vi "RPC Method ThermalChamberController StopModule.vi"(8 "error in (no error)":errorcluster, 11 "gRPC service in":refnum<class "ThermalChamberController.lvclass">) -> (0 "error out":errorcluster, 3 "gRPC service out":refnum<class "ThermalChamberController.lvclass">)   [LabVIEW 2020, in "thermal-chamber-controller_server.lvlib" / "ThermalChamberController.lvclass"]
uses:
  ThermalChamberController.lvclass
  ThermalChamberController.lvclass/ThermalChamberController.ctl
  Program Files (x86)/National Instruments/LabVIEW 2020/examples/DQMH Consortium/DQMH Fundamentals - Thermal Chamber/Libraries/Thermal Chamber Controller_DQMH/Thermal Chamber Controller_DQMH.lvlib
  RPC Messages/lv_python_grpc_webui_demo_v1_Empty.ctl
  thermal-chamber-controller_server.lvlib
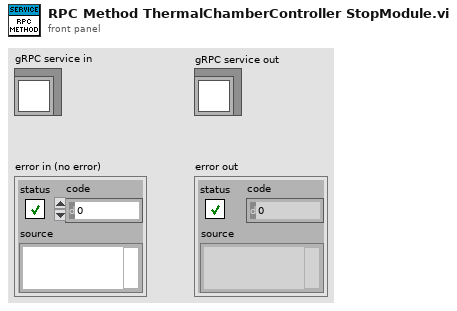
[diagram p1: front panel]
types:
  T1 = typedef "thermal-chamber-controller_server.lvlib/lv_python_grpc_webui_demo_v1_Empty.ctl" = cluster{"void":string}
  T2 = typedef "thermal-chamber-controller_server.lvlib/ThermalChamberController.lvclass/Server Internal UEs.ctl" = cluster{"ThermalChamberController StartModule Internal UE":refnum<user-event>, "ThermalChamberController ShowModulePanel Internal UE":refnum<user-event>, "ThermalChamberController HideModulePanel Internal UE":refnum<user-event>, "ThermalChamberController StopModule Internal UE":refnum<user-event>, "ThermalChamberController UpdateSetPoint Internal UE":refnum<user-event>, "ThermalChamberController UpdateRampRate Internal UE":refnum<user-event>, "ThermalChamberController UpdateHeaterState Internal UE":refnum<user-event>, "ThermalChamberController SubscribeChamberStatusUpdated Internal UE":refnum<user-event>, "ThermalChamberController SubscribeSetPointUpdated Internal UE":refnum<user-event>, "ThermalChamberController SubscribeRampRateUpdated Internal UE":refnum<user-event>, "ThermalChamberController SubscribeHeaterStateUpdated Internal UE":refnum<user-event>}
  T3 = typedef "thermal-chamber-controller_server.lvlib/ThermalChamberController.lvclass/Server gRPC UEs.ctl" = cluster{"ThermalChamberController StartModule gRPC UE":refnum<user-event>, "ThermalChamberController ShowModulePanel gRPC UE":refnum<user-event>, "ThermalChamberController HideModulePanel gRPC UE":refnum<user-event>, "ThermalChamberController StopModule gRPC UE":refnum<user-event>, "ThermalChamberController UpdateSetPoint gRPC UE":refnum<user-event>, "ThermalChamberController UpdateRampRate gRPC UE":refnum<user-event>, "ThermalChamberController UpdateHeaterState gRPC UE":refnum<user-event>, "ThermalChamberController SubscribeChamberStatusUpdated gRPC UE":refnum<user-event>, "ThermalChamberController SubscribeSetPointUpdated gRPC UE":refnum<user-event>, "ThermalChamberController SubscribeRampRateUpdated gRPC UE":refnum<user-event>, "ThermalChamberController SubscribeHeaterStateUpdated gRPC UE":refnum<user-event>}
  T4 = typedef "grpc-lvsupport-release.lvlib/grpcId.ctl" = u64
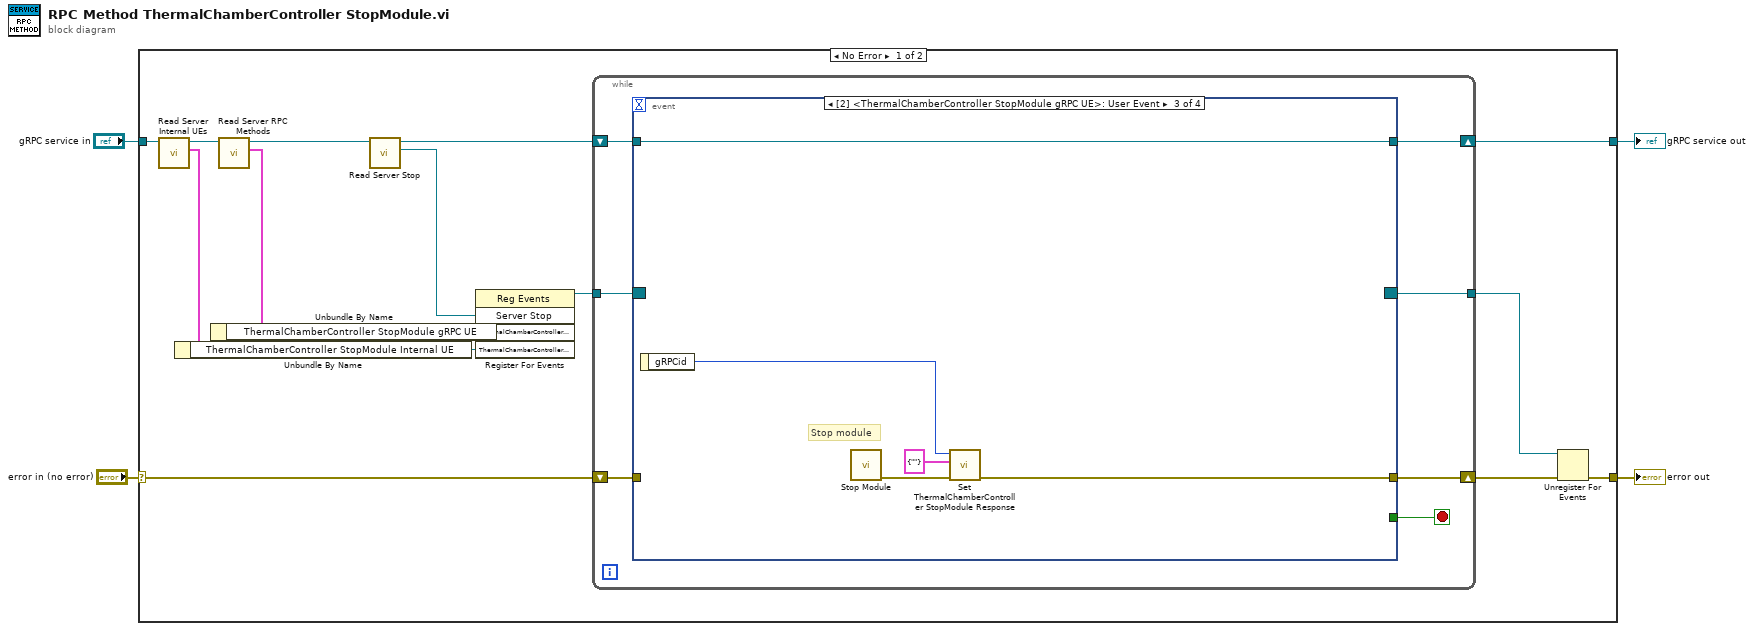
[diagram p0: block diagram]
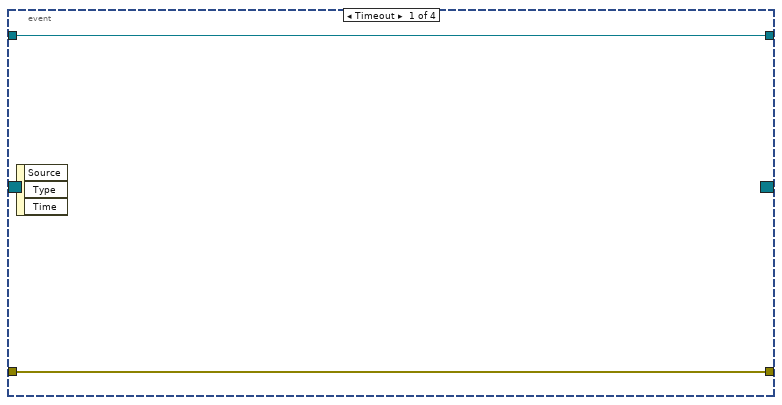
[diagram p2: hidden frame]
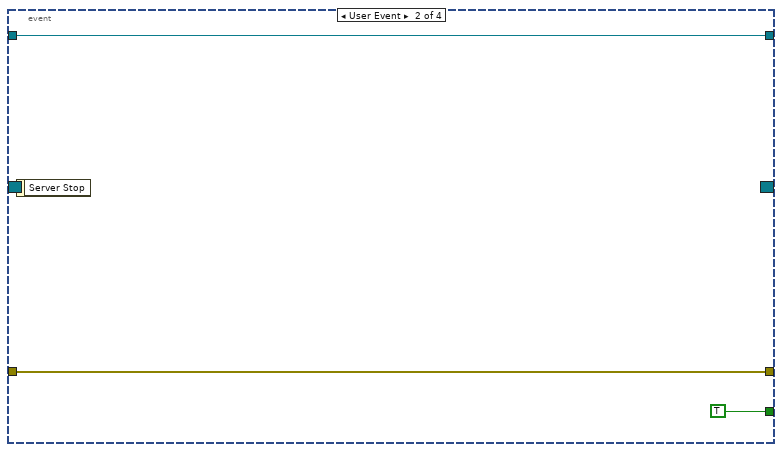
[diagram p3: hidden frame]
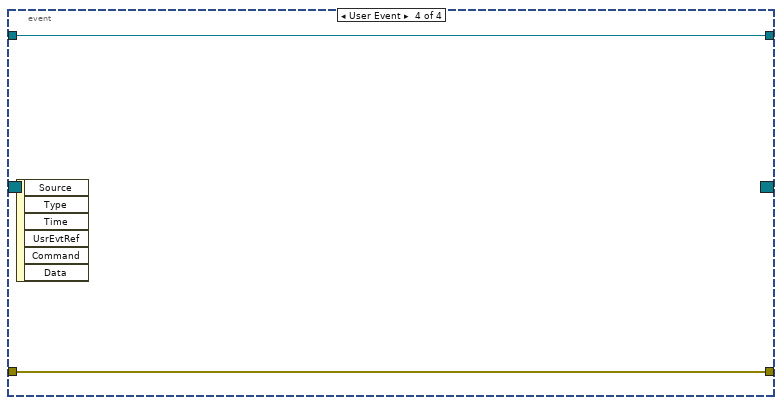
[diagram p4: hidden frame]
diagram:
  n1 = case shown="No Error" "error in (no error)" {
    selector: "error in (no error)" -> [w15 w40]
    tunnel: [w13 w40] -> w3
    tunnel: "gRPC service in" -> [w17 w39]
    tunnel: [w5 w39] -> w1
    frame No Error {
      n2 = call "Read Server Internal UEs.vi"("gRPC service in"=w17) -> ("Server Internal UEs"=w9:T2, "gRPC service out"=w16:refnum<class "ThermalChamberController.lvclass">)  [unwired: 8 in, 1 out]
      n3 = Unbundle By Name ("Unbundle Internal UE")(w9) -> ("ThermalChamberController StopModule Internal UE"=w8:refnum<user-event>)
      n4 = call "Read Server RPC Methods.vi"("gRPC service in"=w16) -> ("Server RPC Methods"=w11:T3, "gRPC service out"=w6:refnum<class "ThermalChamberController.lvclass">)  [unwired: 8 in, 1 out]
      n5 = Unbundle By Name ("Unbundle gRPC UE")(w11) -> ("ThermalChamberController StopModule gRPC UE"=w10:refnum<user-event>)
      n6 = call-dynamic "Read Server Stop.vi"("gRPC service in"=w6) -> ("Server Stop"=w19:refnum<user-event>, "gRPC service out"=w7:refnum<class "ThermalChamberController.lvclass">)  [unwired: 8 in, 1 out]
      n7 = register-events(w19, w10, w8) -> (reference out=w18:refnum<event-registration>)  [unwired: 2 in, 1 out]
      n8 = while {
        tunnel: w18 -> [w26]
        tunnel: [w22] -> w12
        shift-right: [w23] -> w14
        shift-left: w15 -> [w24]
        shift-right: [w20] -> w5
        shift-left: w7 -> [w21]
        stop <- w25 stop-if-true
        n9 = event "RPC Method Event Structure" shown="[2] <ThermalChamberController StopModule gRPC UE>: User Event" {
          selector: w26 -> [_ _ _ _]
          dyn-events: [_ _ _ _] -> w22
          timeout: _ -> [_ _ _ _]
          tunnel: [_ TRUE _ _] -> w25
          tunnel: w24 -> [w28 w30 _ w38]
          tunnel: [w28 w30 w33 w38] -> w23
          tunnel: w21 -> [w27 w29 w36 w37]
          tunnel: [w27 w29 w36 w37] -> w20
          event Timeout {
            n10 = event-data() -> ()  [unwired: 1 in, 3 out]
          }
          event User Event {
            n11 = event-data() -> ()  [unwired: 1 in, 1 out]
          }
          event User Event {
            # "Stop module"
            n12 = event-data() -> ("gRPCid"=w35:T4)  [unwired: 1 in]
            n13 = call "Stop Module.vi"() -> ("error out"=w34:errorcluster)  [unwired: 11 in]
            n14 = call "Set ThermalChamberController StopModule Response.vi"("error in (no error)"=w34, "Message Data"=T1 {"void"=""}, "gRPCid in"=w35) -> ("error out"=w33:errorcluster)  [unwired: 8 in]
          }
          event User Event {
            n15 = event-data() -> ()  [unwired: 1 in, 6 out]
          }
        }
      }
      n16 = Unregister For Events(event registration refnum=w12, error in=w14) -> (error out=w13:errorcluster)
    }
    frame Error {
    }
  }
  "error out" <- w3
  "gRPC service out" <- w1
